vi "VIH - CHM Project - HHP Support - Get Key.vi"(7 "Section":string, 8 "error in":errorcluster, 10 "Key":string, 11 "queue":T1) -> (0 "error out":errorcluster, 1 "Value":string, 2 "dup Key":string, 3 "dup queue":T1)   [LabVIEW 2014]
doc: "::: VI Helpeks :::\nCopyright (c) 2000-2026 Konstantin Shifershteyn. All rights reserved."
uses:
  VIH - CHM Project - HHP Support - Queue Refnum.ctl
  VIH - CHM Project - HHP Support - Config Data Cluster.ctl
panel:
  # "VI Helpeks\nCopyright (c) 2012-2026 Konstantin Shifershteyn"
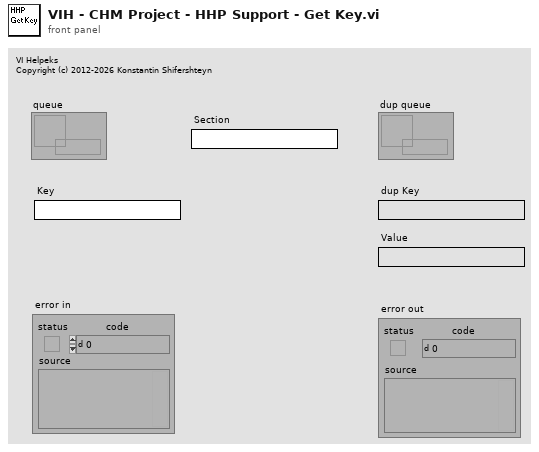
[diagram p1: front panel]
types:
  T1 = typedef "VIH - CHM Project - HHP Support - Queue Refnum.ctl" = refnum<queue>
  T2 = typedef "VIH - CHM Project - HHP Support - Config Data Cluster.ctl" = cluster{"Fille path":path, "sections":cluster{"Sec name":string, "key-values":string[][]}[]}
  T3 = cluster{"Sec name":string, "key-values":string[][]}[]
  T4 = cluster{"Sec name":string, "key-values":string[][]}
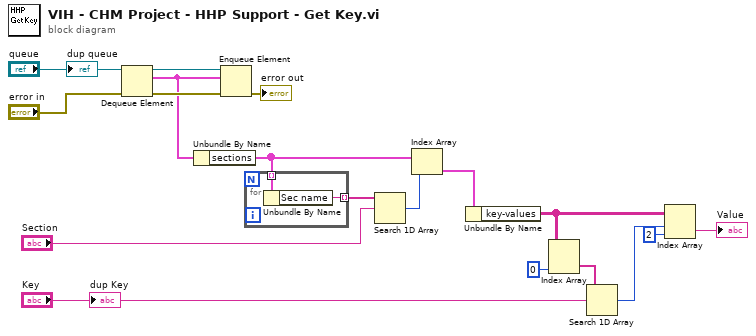
[diagram p0: block diagram]
diagram:
  n1 = Dequeue Element(queue="queue", error in (no error)="error in") -> (queue out=w18:T1, element=w1:T2, error out=w15:errorcluster)  [unwired: 1 in, 1 out]
  n2 = Unbundle By Name(w1) -> ("sections"=w9:T3)
  n3 = Enqueue Element(queue=w18, element=w1, error in (no error)=w15) -> (error out=→"error out":errorcluster)  [unwired: 1 in, 2 out]
  n4 = for {
    tunnel: w9 -> [w20] mode=indexing
    tunnel: [w19] -> w11 mode=indexing
    n5 = Unbundle By Name(w20) -> ("Sec name"=w19:string)
  }
  n6 = Search 1D Array(1D array=w11, element="Section") -> (index of element=w10:i32)  [unwired: 1 in]
  n7 = Index Array(array=w9, index=w10) -> (element=w6:T4)
  n8 = Unbundle By Name(w6) -> ("key-values"=w5:string[][])
  n9 = Index Array(array=w5, index (col)=0 ("disabled index (col)")) -> (element=w7:string[])  [unwired: 1 in]
  n10 = Search 1D Array(1D array=w7, element="Key") -> (index of element=w4:i32)  [unwired: 1 in]
  n11 = Index Array(array=w5, index (row)=w4, index (col)=2 ("disabled index (col)")) -> (element=→"Value":string)
  "dup queue" <- "queue"
  "dup Key" <- "Key"
